vi "C_WS_BuildFrame.vi"(8 "error in (no error)":errorcluster, 10 "opcode":u8=2, 11 "payload":u8[](array[numeric]) format="%.0x") -> (0 "error out":errorcluster, 3 "frame":u8[](array[numeric]) format="%.0x")   [LabVIEW 2021, in "CANsub_C.lvlib"]
doc: "Builds one masked WebSocket client frame (FIN set) around a payload, ready for TCP Write. opcode: 2 binary, 8 close, 9 ping, 10 pong. Fixed mask 12 34 56 78 (the device does not check it)."
uses:
  CANsub_C.lvlib
  codec_vis/CANsub_Codec.lvlib
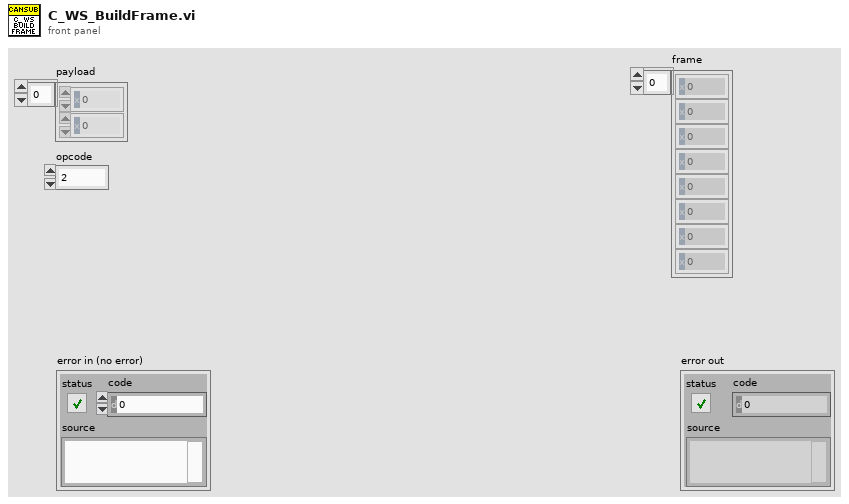
[diagram p1: front panel]
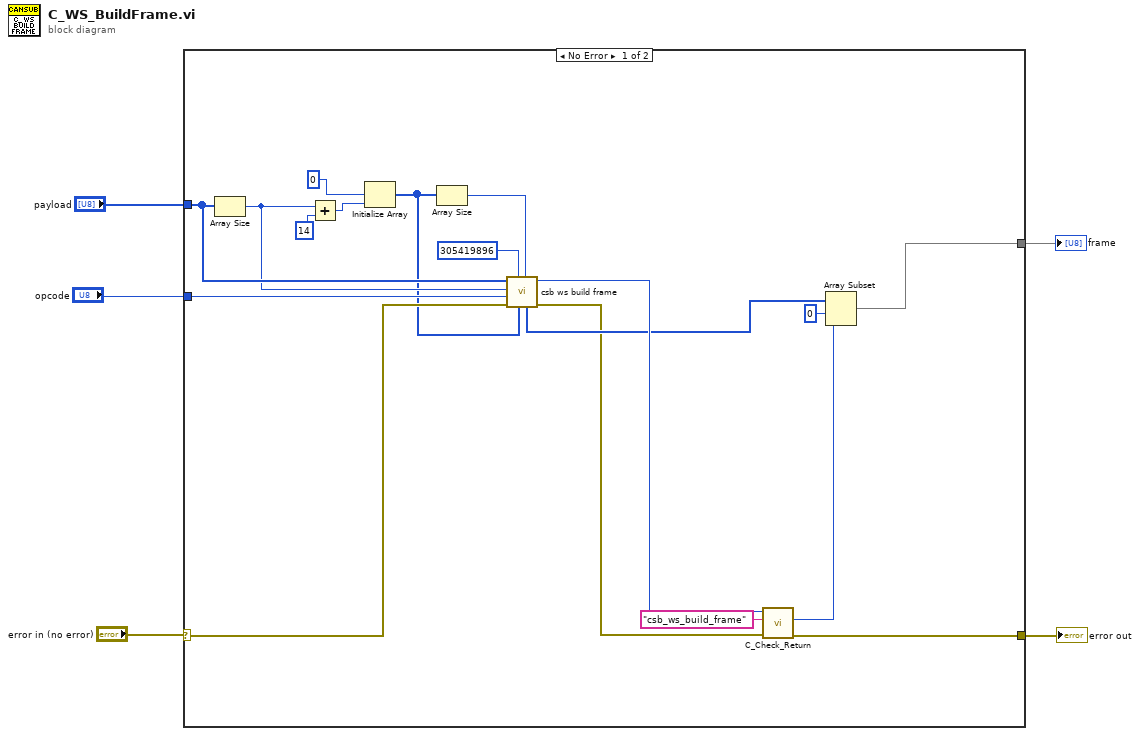
[diagram p0: block diagram]
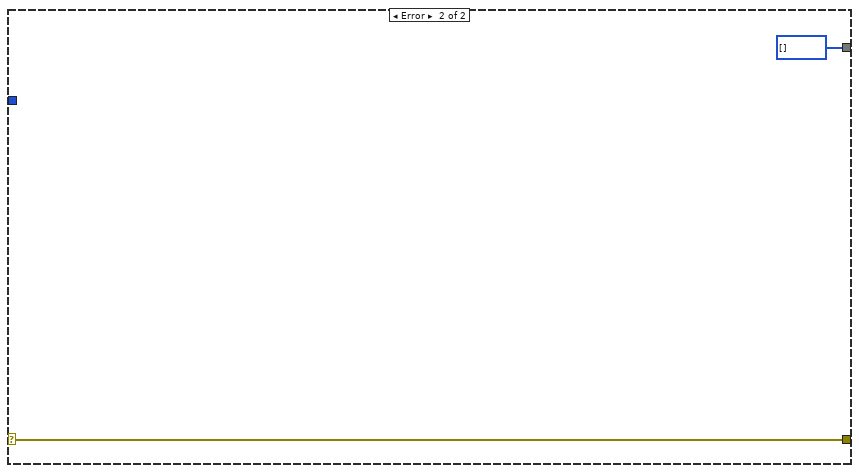
[diagram p2: hidden frame]
diagram:
  n1 = case shown="No Error" "error in (no error)" {
    selector: "error in (no error)" -> [w10 w24]
    tunnel: [w12 u8[] [] ("frame")] -> w4
    tunnel: [w9 w24] -> w3
    tunnel: "payload" -> [w21 _]
    tunnel: "opcode" -> [w19 _]
    frame No Error {
      n2 = Array Size(array=w21) -> (size(s)=w20:i32)
      n3 = Add(x=w20, y=14) -> (x+y=w17:i32)
      n4 = Initialize Array(u8 0, w17) -> (w7:u8[])
      n5 = Array Size(array=w7) -> (size(s)=w6:i32)
      n6 = call "csb ws build frame.vi"("frame_cap"=w6, "frame"=w7, "mask"=u32 305419896, "error in (no error)"=w10, "opcode"=w19, "len"=w20, "payload"=w21) -> ("error out"=w11:errorcluster, "function return"=w16:i32, "frame out"=w15:u8[])  [unwired: 2 in]
      n7 = call "C_Check_Return.vi"("error in (no error)"=w11, "function name"="csb_ws_build_frame", "function return"=w16) -> ("error out"=w9:errorcluster, "length"=w13:i32)  [unwired: 6 in, 1 out]
      n8 = Array Subset(array=w15, index=0, length=w13) -> (w12:u8[])
    }
    frame Error {
    }
  }
  "error out" <- w3
  "frame" <- w4
